vi "work2_Cooker_Module.vi"() -> ()   [LabVIEW 2026]
panel:
  in  "number":i32
  in  "Burgers":bool
  in  "Meal":bool
  in  "stop":bool
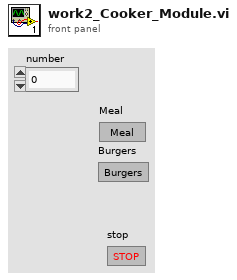
[diagram p1: front panel]
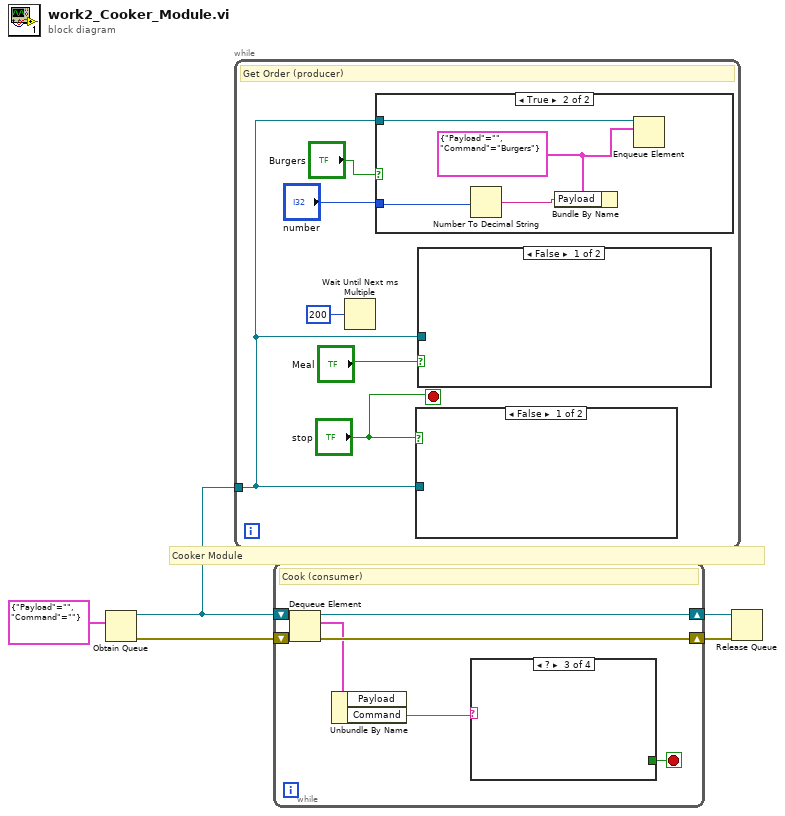
[diagram p0: block diagram]
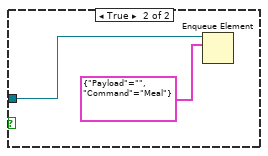
[diagram p3: hidden frame]
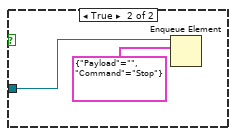
[diagram p4: hidden frame]
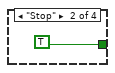
[diagram p6: hidden frame]
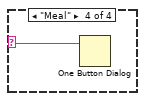
[diagram p7: hidden frame]
diagram:
  # "Cooker Module"
  n1 = Obtain Queue(element data type=cluster{"Payload":string, "Command":string} {"Payload"="", "Command"=""}) -> (queue out=w2:refnum<queue>, error out=w4:errorcluster)  [unwired: 4 in, 1 out]
  n2 = while {
    tunnel: w2 -> [w8]
    stop <- "stop" stop-if-true
    # "Get Order (producer)"
    n3 = Wait Until Next ms Multiple(millisecond multiple=u32 200) -> ()  [unwired: 1 out]
    n4 = case shown="True" "Burgers" {
      tunnel: w8 -> [_ w15]
      tunnel: "number" -> [_ w12]
      frame False {
      }
      frame True {
        w14 = cluster{"Payload":string, "Command":string} {"Payload"="", "Command"="Burgers"} ("element")
        n5 = Number To Decimal String(number=w12) -> (decimal integer string=w13:string)  [unwired: 1 in]
        n6 = Bundle By Name(cluster=w14, "Payload"=w13) -> ()  [unwired: 1 out]
        n7 = Enqueue Element(queue=w15, element=w14) -> ()  [unwired: 2 in, 3 out]
      }
    }
    n8 = case shown="False" "stop" {
      tunnel: w8 -> [_ w19]
      frame False {
      }
      frame True {
        n9 = Enqueue Element(queue=w19, element=cluster{"Payload":string, "Command":string} {"Payload"="", "Command"="Stop"}) -> ()  [unwired: 2 in, 3 out]
      }
    }
    n10 = case shown="False" "Meal" {
      tunnel: w8 -> [_ w17]
      frame False {
      }
      frame True {
        n11 = Enqueue Element(queue=w17, element=cluster{"Payload":string, "Command":string} {"Payload"="", "Command"="Meal"}) -> ()  [unwired: 2 in, 3 out]
      }
    }
  }
  n12 = while {
    shift-right: [w24] -> w3
    shift-left: w4 -> [w25]
    shift-right: [w26] -> w5
    shift-left: w2 -> [w23]
    stop <- w20 stop-if-true
    # "Cook (consumer)"
    n13 = Dequeue Element(queue=w23, error in (no error)=w25) -> (queue out=w26:refnum<queue>, element=w22:cluster{"Payload":string, "Command":string}, error out=w24:errorcluster)  [unwired: 1 in, 1 out]
    n14 = Unbundle By Name(w22) -> ("Command"=w21:string)  [unwired: 1 out]
    n15 = case w21 {
      selector: w21 -> [_ _ _ w28]
      tunnel: [_ TRUE _ _] -> w20
      frame Default {
      }
      frame "Stop" {
      }
      frame ? {
      }
      frame "Meal" {
        n16 = One Button Dialog(message=w28) -> ()  [unwired: 1 in, 1 out]
      }
    }
  }
  n17 = Release Queue(queue=w5, error in (no error)=w3) -> ()  [unwired: 1 in, 3 out]
